vi "Kill Service.vi"(8 "error in":errorcluster, 11 "full exe name":string) -> (0 "error out":errorcluster)   [LabVIEW 2021, in "MeasurementServerTests.lvlib"]
uses:
  MeasurementServerTests.lvlib
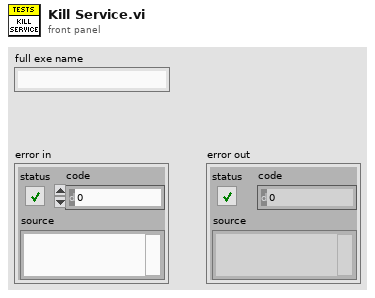
[diagram p1: front panel]
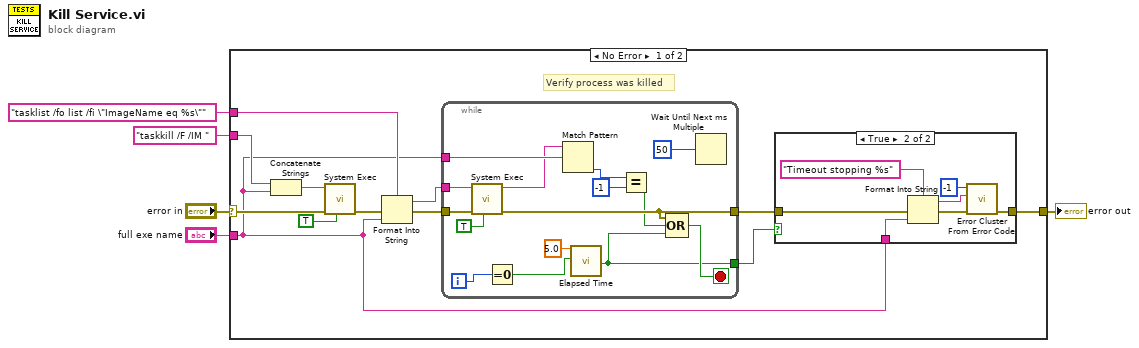
[diagram p0: block diagram]
diagram:
  n1 = case shown="No Error" "error in" {
    selector: "error in" -> [w10 w41]
    tunnel: "taskkill /F /IM " -> [w17 _]
    tunnel: "tasklist /fo list /fi \"ImageName eq %s\"" -> [w12 _]
    tunnel: "full exe name" -> [w6 _]
    tunnel: [w8 w41] -> w1
    frame No Error {
      # "Verify process was killed"
      n2 = Concatenate Strings(w17, w6) -> (w16:string)
      n3 = call <vilib>:"System Exec.vi"("run minimized? (F)"=TRUE, "error in (no error)"=w10, "command line"=w16) -> ("error out"=w14:errorcluster)  [unwired: 5 in, 3 out]
      n4 = Format Into String(format string=w12, error in=w14, w6) -> (resulting string=w11:string, error out=w13:errorcluster)  [unwired: 1 in]
      n5 = while {
        tunnel: w6 -> [w39]
        tunnel: w11 -> [w36]
        tunnel: w13 -> [w40]
        tunnel: [w32] -> w9
        tunnel: [w28] -> w7
        i -> [w27]
        stop <- w30 stop-if-true
        n6 = call <vilib>:"System Exec.vi"("run minimized? (F)"=TRUE, "error in (no error)"=w40, "command line"=w36) -> ("error out"=w32:errorcluster, "standard output"=w35:string)  [unwired: 5 in, 2 out]
        n7 = Equal To 0?(x=w27) -> (x = 0?=w26:bool)
        n8 = Match Pattern(string=w35, regular expression=w39) -> (offset past match=w38:i32)  [unwired: 1 in, 3 out]
        n9 = call "Elapsed Time"("Time Target (s)"=5.0, "Reset"=w26) -> ("Time has Elapsed"=w28:bool)  [unwired: 10 in, 7 out]
        n10 = Equal?(x=w38, y=-1) -> (x = y?=w31:bool)
        n11 = Compound Arithmetic op=OR(w32, w31, w28) -> (w30:bool)
        n12 = Wait Until Next ms Multiple(millisecond multiple=u32 50) -> ()  [unwired: 1 out]
      }
      n13 = case shown="True" w7 {
        tunnel: w9 -> [w18 w23]
        tunnel: [w18 w25] -> w8
        tunnel: w6 -> [_ w21]
        frame False {
        }
        frame True {
          n14 = Format Into String(format string="Timeout stopping %s", error in=w23, w21) -> (resulting string=w19:string, error out=w22:errorcluster)  [unwired: 1 in]
          n15 = call <vilib>:"Error Cluster From Error Code.vi"("error in (no error)"=w22, "error message (\"\")"=w19, "error code (0)"=-1) -> ("error out"=w25:errorcluster)  [unwired: 6 in]
        }
      }
    }
    frame Error {
    }
  }
  "error out" <- w1
